vi "character_condition.vi"() -> ()   [LabVIEW 2021]
panel:
  out "string condition":bool[](array[boolean])
  out "int condition":bool[](array[boolean])
  out "char condition":bool[](array[boolean])
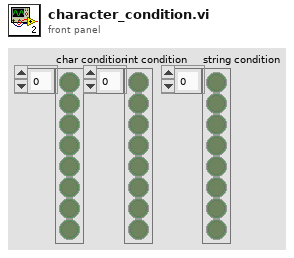
[diagram p1: front panel]
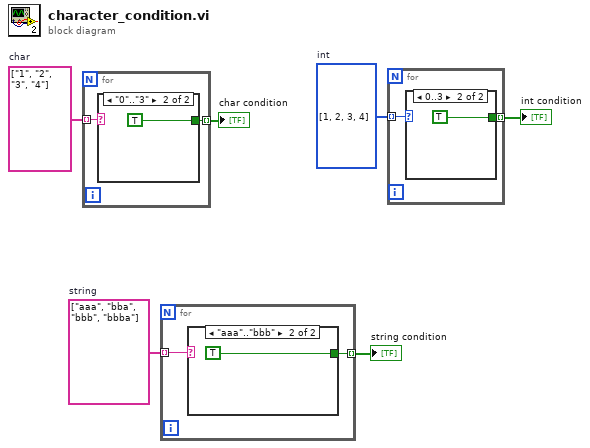
[diagram p0: block diagram]
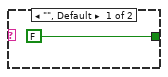
[diagram p2: hidden frame]
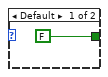
[diagram p3: hidden frame]
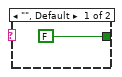
[diagram p4: hidden frame]
diagram:
  w1 = string[] ["aaa", "bba", "bbb", "bbba"]  # string
  w3 = i32[] [1, 2, 3, 4]  # int
  w6 = string[] ["1", "2", "3", "4"]  # char
  n1 = for {
    tunnel: w6 -> [w8] mode=indexing
    tunnel: [w7] -> w5 mode=indexing
    n2 = case shown="\"0\"..\"3\"" w8 {
      tunnel: [FALSE TRUE] -> w7
      frame "", Default {
      }
      frame "0".."3" {
      }
    }
  }
  "char condition" <- w5
  n3 = for {
    tunnel: w1 -> [w12] mode=indexing
    tunnel: [w11] -> w2 mode=indexing
    n4 = case shown="\"aaa\"..\"bbb\"" w12 {
      tunnel: [FALSE TRUE] -> w11
      frame "", Default {
      }
      frame "aaa".."bbb" {
      }
    }
  }
  "string condition" <- w2
  n5 = for {
    tunnel: w3 -> [w16] mode=indexing
    tunnel: [w15] -> w4 mode=indexing
    n6 = case shown="0..3" w16 {
      tunnel: [FALSE TRUE] -> w15
      frame Default {
      }
      frame 0..3 {
      }
    }
  }
  "int condition" <- w4
